vi "translate error code.vi"(8 "error in (no error)":errorcluster, 10 "error code":u32 format="%x") -> (0 "error out":errorcluster)   [LabVIEW 2024, in "atsj peakcan basic.lvlib"]
doc: "Converts an <b>error code</b> into an error cluster and merges it with the <b>error in</b> cluster."
uses:
  atsj peakcan basic.lvlib
  <vilib>/Utility/error.llb/whitespace.ctl
  <vilib>/Utility/error.llb/Trim Whitespace One-Sided.vi
  support/x64/PCANBasic.dll
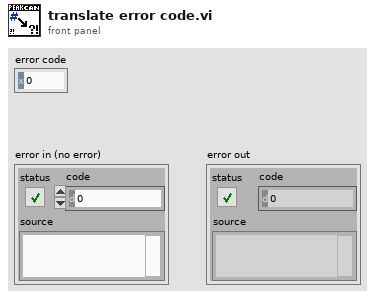
[diagram p1: front panel]
types:
  T1 = typedef "whitespace.ctl" = u16
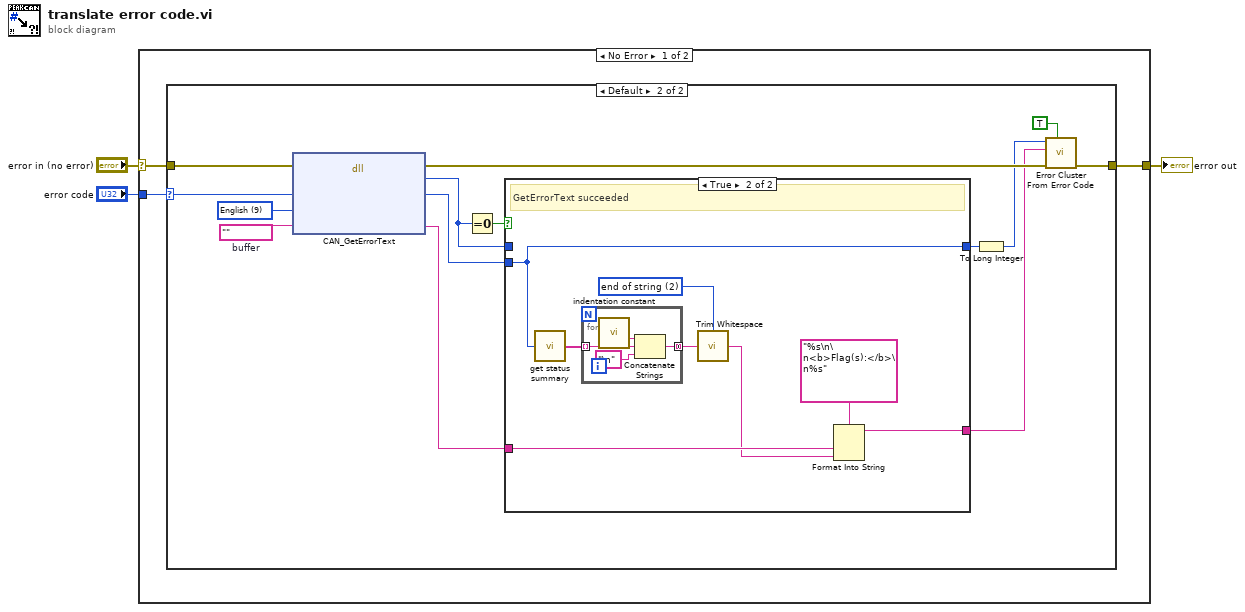
[diagram p0: block diagram]
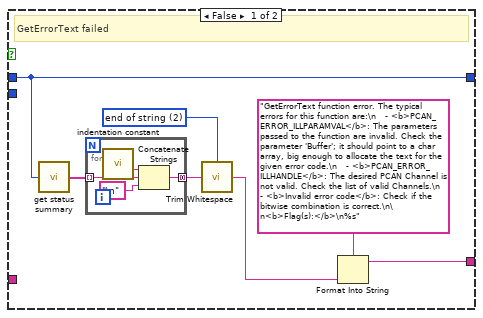
[diagram p3: hidden frame]
diagram:
  n1 = case shown="No Error" "error in (no error)" {
    selector: "error in (no error)" -> [w4 w45]
    tunnel: "error code" -> [w6 _]
    tunnel: [w5 w45] -> w1
    frame No Error {
      n2 = case shown="Default" w6 {
        selector: w6 -> [_ w9]
        tunnel: [w7 w15] -> w5
        tunnel: w4 -> [w7 w21]
        frame 0 {
        }
        frame Default {
          w18 = ""  # buffer
          w19 = u16 9 items=["System"=0, "German"=7, "English"=9, "Spanish"=10, "French"=12, "Italian"=16]
          n3 = dll-call lib="C:/atsj/plateau/atsj-peakcan-basic-for-labview/src/support/x64/PCANBasic.dll" fn="CAN_GetErrorText"(error in=w21, "Error"=w9, "Language"=w19, "Buffer"=w18) -> (error out=w20:errorcluster, "return type"=w13:u32, "Error"=w8:u32, "Buffer"=w16:string)  [unwired: 3 in, 1 out]
          n4 = Equal To 0?(x=w13) -> (x = 0?=w10:bool)
          n5 = case shown="True" w10 {
            tunnel: w8 -> [_ w33]
            tunnel: [w27 w38] -> w17
            tunnel: w16 -> [_ w39]
            tunnel: [w23 w33] -> w12
            tunnel: w13 -> [w23 _]
            frame False {
              w24 = T1 2 items=["both", "start of string", "end of string"]
              # "GetErrorText failed"
              n6 = call "get status summary.vi"("status code"=w23) -> ("flag names"=w26:string[])
              n7 = for {
                tunnel: w26 -> [w32] mode=indexing
                tunnel: [w30] -> w25 mode=concatenating
                n8 = call "indentation constant.vi"() -> ("indentation"=w29:string)
                n9 = Concatenate Strings(w29, w32, "\n") -> (w30:string)
              }
              n10 = call <vilib>:"Trim Whitespace.vi"("string"=w25, "location (both)"=w24) -> ("trimmed string"=w22:string)
              n11 = Format Into String(format string="GetErrorText function error. The typical errors for this function are:\n   - <b>PCAN_ERROR_ILLPARAMVAL</b>: The parameters passed to the function are invalid. Check the parameter 'Buffer'; it should point to a char array, big enough to allocate the text for the given error code.\n   - <b>PCAN_ERROR_ILLHANDLE</b>: The desired PCAN Channel is not valid. Check the list of valid Channels.\n   - <b>Invalid error code</b>: Check if the bitwise combination is correct.\n\n<b>Flag(s):</b>\n%s", w22) -> (resulting string=w27:string)  [unwired: 2 in, 1 out]
            }
            frame True {
              w34 = T1 2 items=["both", "start of string", "end of string"]
              # "GetErrorText succeeded"
              n12 = call "get status summary.vi"("status code"=w33) -> ("flag names"=w37:string[])
              n13 = for {
                tunnel: w37 -> [w44] mode=indexing
                tunnel: [w42] -> w36 mode=concatenating
                n14 = call "indentation constant.vi"() -> ("indentation"=w41:string)
                n15 = Concatenate Strings(w41, w44, "\n") -> (w42:string)
              }
              n16 = call <vilib>:"Trim Whitespace.vi"("string"=w36, "location (both)"=w34) -> ("trimmed string"=w35:string)
              n17 = Format Into String(format string="%s\n\n<b>Flag(s):</b>\n%s", w39, w35) -> (resulting string=w38:string)  [unwired: 2 in, 1 out]
            }
          }
          n18 = To Long Integer(number=w12) -> (32bit integer=w11:i32)
          n19 = call <vilib>:"Error Cluster From Error Code.vi"("show call chain? (False)"=TRUE, "error in (no error)"=w20, "error message (\"\")"=w17, "error code (0)"=w11) -> ("error out"=w15:errorcluster)  [unwired: 5 in]
        }
      }
    }
    frame Error {
    }
  }
  "error out" <- w1
